vi "Write Name.vi"(8 "error in":errorcluster, 10 "Name":string, 11 "Engine in":refnum<class "Engine Parent Editor Node.lvclass">) -> (0 "error out":errorcluster, 3 "Engine out":refnum<class "Engine Parent Editor Node.lvclass">)   [LabVIEW 2013, in "PL Framework Configuration Tool.lvlib" / "Engine Parent Editor Node.lvclass"]
uses:
  Engine Parent Editor Node.lvclass
  <vilib>/NI/Configuration Framework/serializable configuration/NISE_CEF_serializable configuration.lvclass
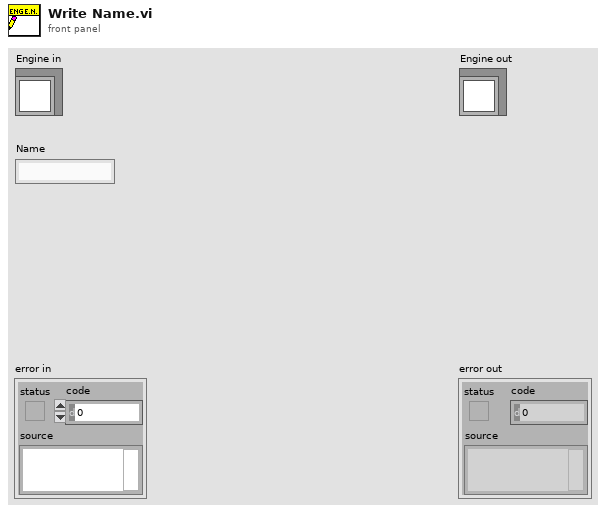
[diagram p1: front panel]
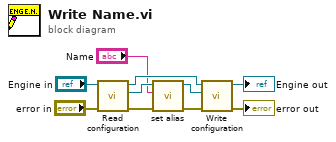
[diagram p0: block diagram]
diagram:
  n1 = call-dynamic "Read configuration.vi"("error in"="error in", "NISE_CEF_serializable node in"="Engine in") -> ("error out"=w5:errorcluster, "configuration"=w4:refnum<class "NISE_CEF_serializable configuration.lvclass">, "NISE_CEF_serializable node out"=w10:refnum<class "Engine Parent Editor Node.lvclass">)  [unwired: 7 in]
  n2 = call <vilib>:"set alias.vi"("error in"=w5, "alias"="Name", "configuration in"=w4) -> ("error out"=w2:errorcluster, "configuration out"=w3:refnum<class "NISE_CEF_serializable configuration.lvclass">)  [unwired: 7 in]
  n3 = call-dynamic "Write configuration.vi"("error in"=w2, "configuration"=w3, "NISE_CEF_serializable node in"=w10) -> ("error out"=→"error out":errorcluster, "NISE_CEF_serializable node out"=→"Engine out":refnum<class "Engine Parent Editor Node.lvclass">)  [unwired: 7 in]
